vi "global names.vi"() -> (1 "dataset RID":string="dataset RID", 2 "API Key":string="nominal api key", 3 "logged channels name":string="Select Channels")   [LabVIEW 2020, in "Nominal-Streamer.lvlib" / "Nominal-Streamer.lvclass"]
uses:
  Nominal-Streamer.lvclass
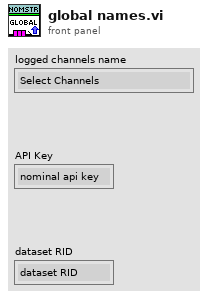
[diagram p1: front panel]
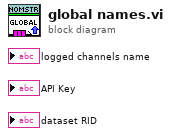
[diagram p0: block diagram]
diagram:
